vi "data to write.vi"(11 "write data":u8[](array[numeric])) -> ()   [LabVIEW 2012]
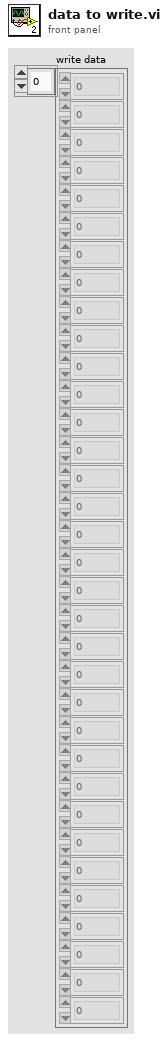
[diagram p1: front panel]
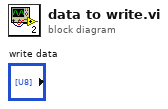
[diagram p0: block diagram]
diagram:
